vi "Save Wave Data.vi"(10 "Time and Data":T3, 11 "Sample Settings":T1={"设备信息"={"初始索引子集"=[], "模拟信号采集通道"="", "数字-供电"="", "数字-光控"="", "光控设备"="", "光电设备分离？"=FALSE, "光谱保存路径"=path "", "环数"=0}, "测量控制"={"测头拿起"=FALSE, "起始保存"=FALSE, "测头供电"=TRUE, "测头出光"=TRUE}, "测量"={"每波长测量次数"=5, "波长"=[0, 0, 0, 0, 0, 0], "起始周期"=0, "起始测量周期"=0}, "等待"={"等待时间(s)"=0.0, "等待方式"=FALSE, "每x周期/点等待"=8, "等待时"=enum."无电无光"}, "校准"={"暗电流校准值初值"=[], "温度校准值"=[0.0, 0.0, 0.0, 0.0, 0.0, 0.0, 0.00013, 0.00013, 0.00013, 0.00013, 0.00013, 0.00013], "校准模式"=enum."逐周期"}, "图表相关"={"文件-时间"=""}, "CSM"={"CSM Name"=""}}) -> ()   [LabVIEW 2026, in "UI-无创.lvlib" / "Logging.lvlib"]
uses:
  Logging.lvlib
  Supports/Time and Data_OP.ctl
  Supports/Sample Settings.ctl
  <vilib>/Utility/file.llb/Write To Spreadsheet File (DBL).vi
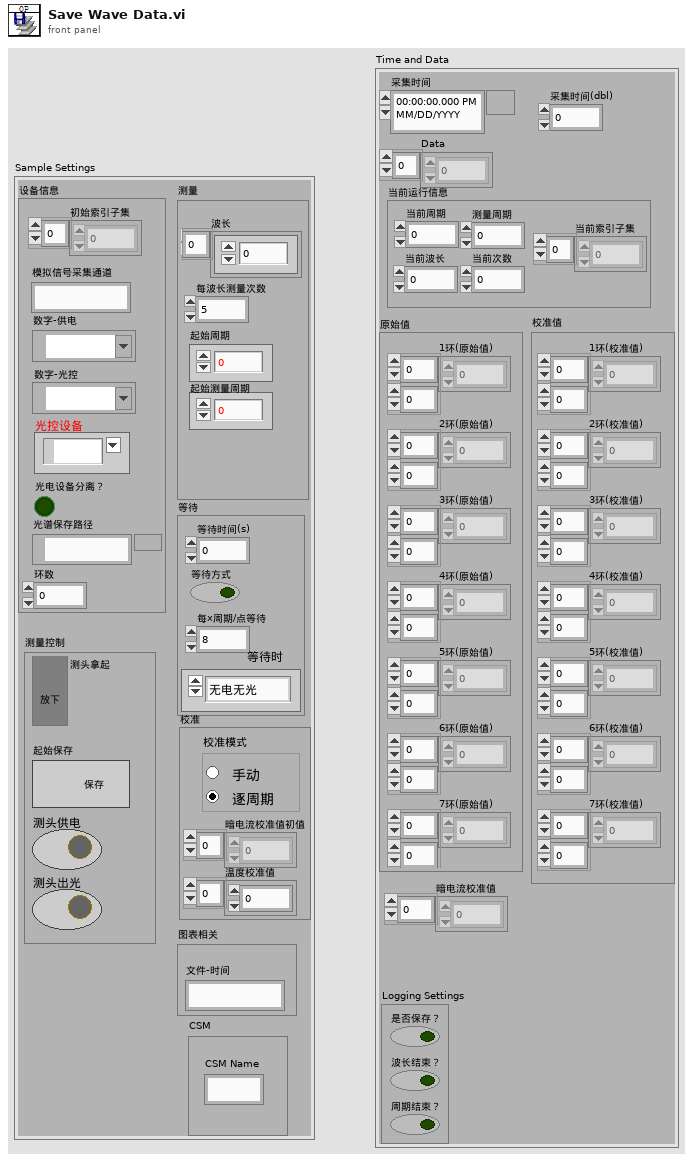
[diagram p1: front panel]
types:
  T1 = typedef "UI-无创.lvlib/Sample Settings.ctl" = cluster{"设备信息":cluster{"初始索引子集":i8[], "模拟信号采集通道":string, "数字-供电":refnum<k21>, "数字-光控":refnum<k21>, "光控设备":tag, "光电设备分离？":bool, "光谱保存路径":path, "环数":u8}, "测量控制":cluster{"测头拿起":bool, "起始保存":bool, "测头供电":bool, "测头出光":bool}, "测量":cluster{"每波长测量次数":i32, "波长":i32[], "起始周期":i32, "起始测量周期":i32}, "等待":cluster{"等待时间(s)":dbl, "等待方式":bool, "每x周期/点等待":i32, "等待时":enum16{"无电无光", "有电无光", "无电有光", "有电有光"}}, "校准":cluster{"暗电流校准值初值":dbl[], "温度校准值":dbl[], "校准模式":T2}, "图表相关":cluster{"文件-时间":string}, "CSM":cluster{"CSM Name":string}}
  T2 = typedef "UI-无创.lvlib/暗电流校准模式.ctl" = enum32{"手动", "逐周期"}
  T3 = typedef "UI-无创.lvlib/Time and Data_OP.ctl" = cluster{"采集时间":timestamp, "采集时间(dbl)":dbl, "Data":dbl[], "当前运行信息":cluster{"当前周期":i32, "当前次数":i32, "测量周期":i32, "当前索引子集":i8[], "当前波长":i32}, "暗电流校准值":dbl[], "Logging Settings":cluster{"是否保存？":bool, "波长结束？":bool, "周期结束？":bool}, "原始值":cluster{"1环(原始值)":dbl[][], "2环(原始值)":dbl[][], "3环(原始值)":dbl[][], "4环(原始值)":dbl[][], "5环(原始值)":dbl[][], "6环(原始值)":dbl[][], "7环(原始值)":dbl[][]}, "校准值":cluster{"1环(校准值)":dbl[][], "2环(校准值)":dbl[][], "3环(校准值)":dbl[][], "4环(校准值)":dbl[][], "5环(校准值)":dbl[][], "6环(校准值)":dbl[][], "7环(校准值)":dbl[][]}}
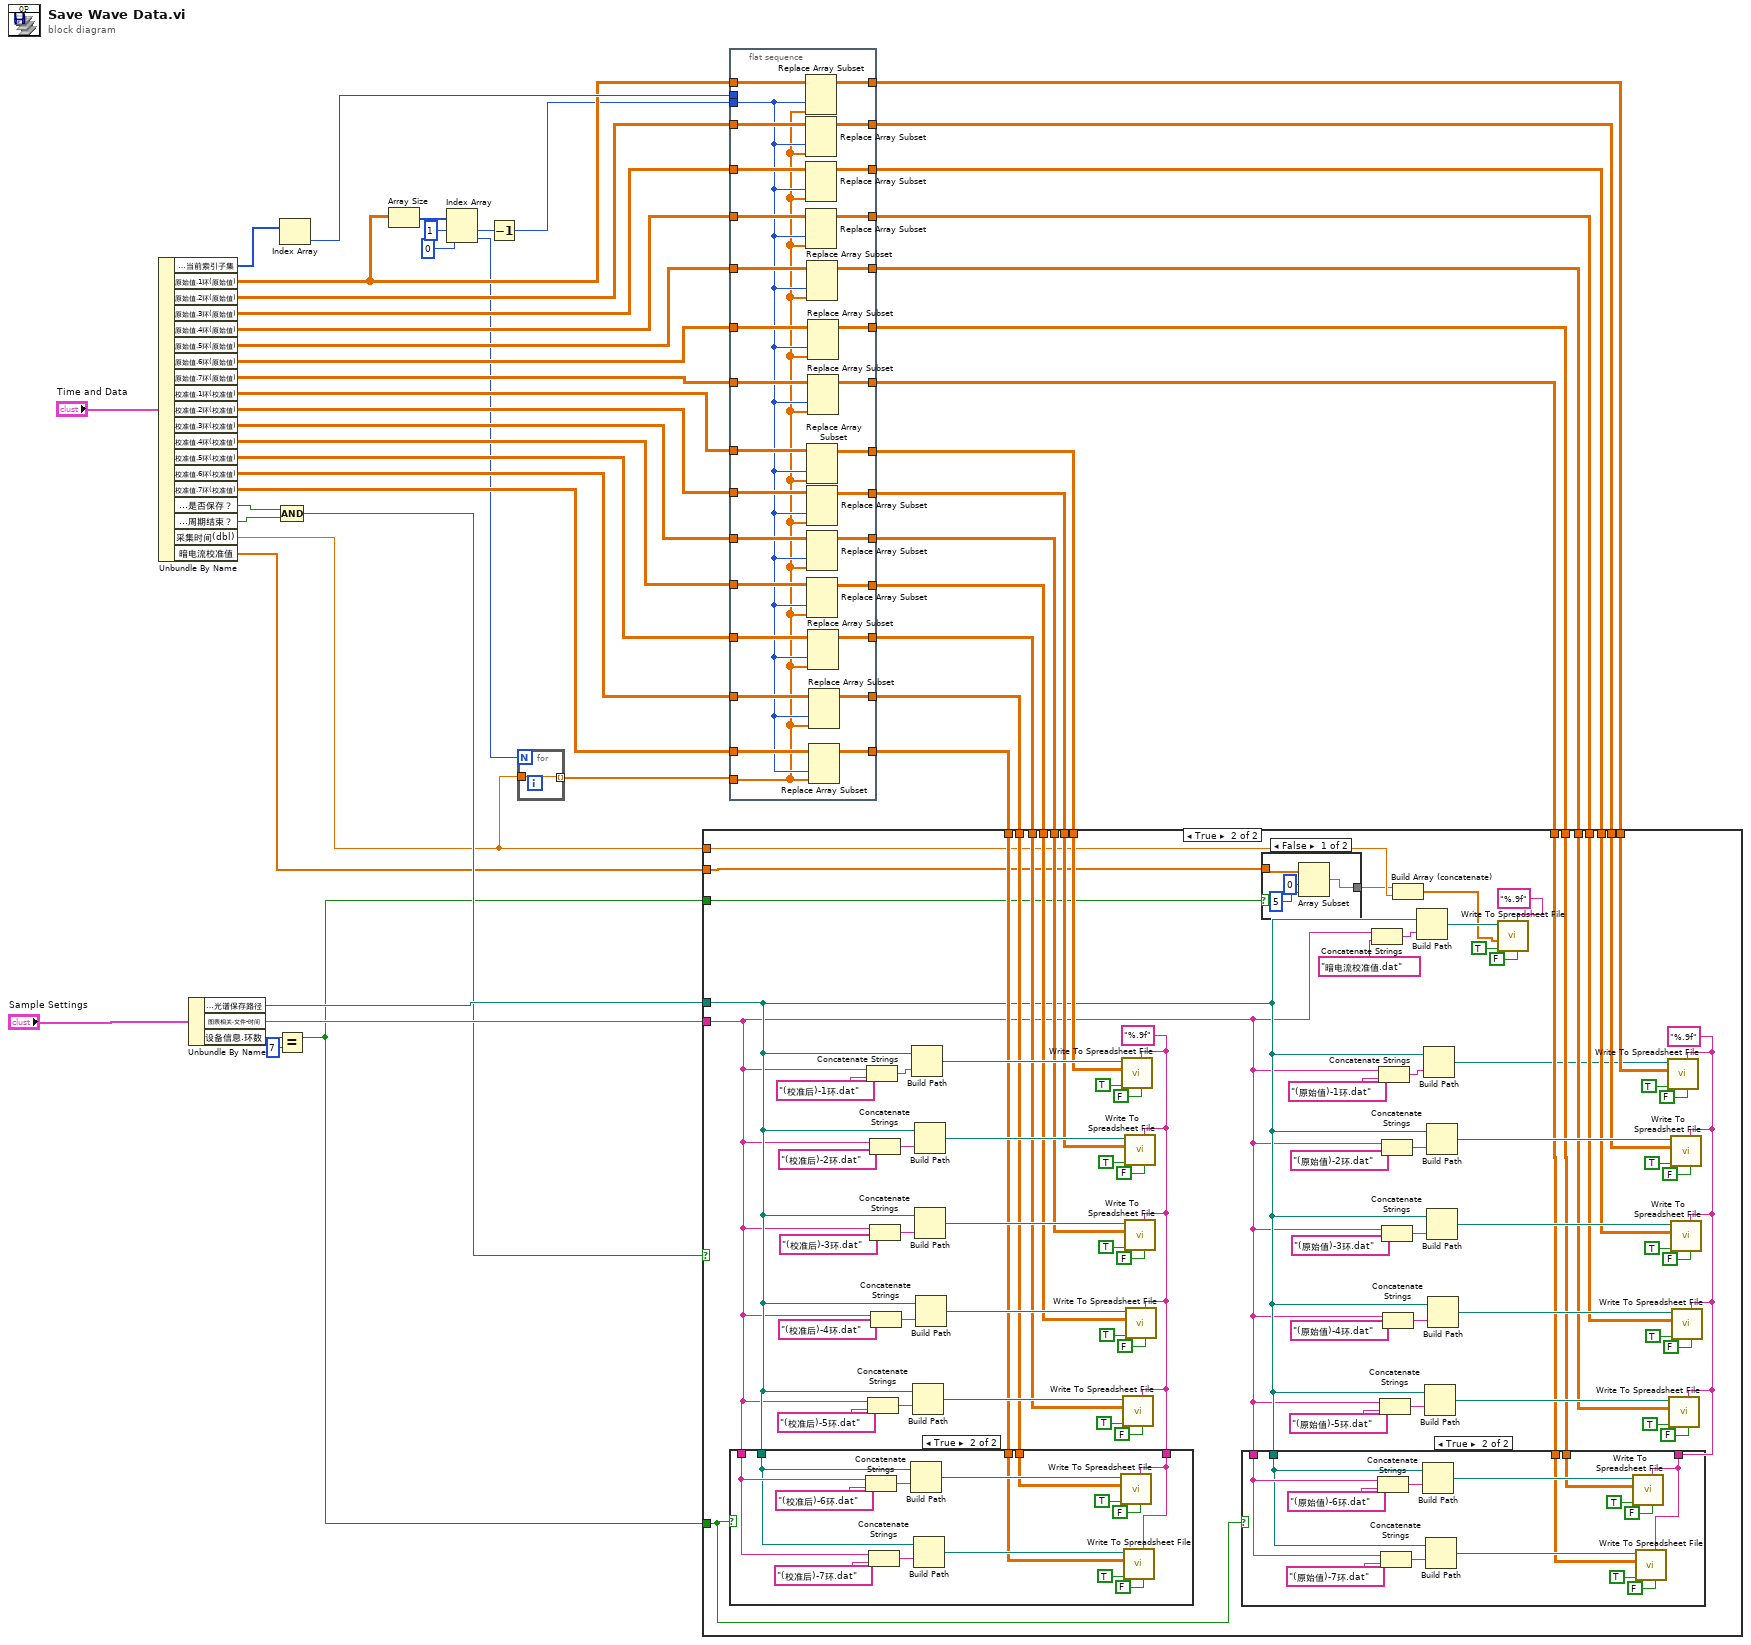
[diagram p0: block diagram]
diagram:
  n1 = Unbundle By Name("Time and Data") -> ("当前运行信息.当前索引子集"=w39:i8[], "原始值.1环(原始值)"=w37:dbl[][], "原始值.2环(原始值)"=w43:dbl[][], "原始值.3环(原始值)"=w42:dbl[][], "原始值.4环(原始值)"=w34:dbl[][], "原始值.5环(原始值)"=w33:dbl[][], "原始值.6环(原始值)"=w32:dbl[][], "原始值.7环(原始值)"=w31:dbl[][], "校准值.1环(校准值)"=w30:dbl[][], "校准值.2环(校准值)"=w28:dbl[][], "校准值.3环(校准值)"=w29:dbl[][], "校准值.4环(校准值)"=w27:dbl[][], "校准值.5环(校准值)"=w26:dbl[][], "校准值.6环(校准值)"=w41:dbl[][], "校准值.7环(校准值)"=w40:dbl[][], "Logging Settings.是否保存？"=w45:bool, "Logging Settings.周期结束？"=w46:bool, "采集时间(dbl)"=w6:dbl, "暗电流校准值"=w9:dbl[])
  n2 = Unbundle By Name("Sample Settings") -> ("设备信息.光谱保存路径"=w48:path, "图表相关.文件-时间"=w47:string, "设备信息.环数"=w8:u8)
  n3 = Equal?(x=w8, y=u8 7) -> (x = y?=w2:bool)
  n4 = Index Array(array=w39) -> (element=w38:i8)  [unwired: 1 in]
  n5 = Compound Arithmetic op=AND ("复合运算")(w45, w46) -> (w44:bool)
  n6 = Array Size(array=w37) -> (size(s)=w36:i32[])
  n7 = Index Array(array=w36, index #1=1 ("索引"), index #2=0 ("索引")) -> (element #1=w10:i32, element #2=w3:i32)
  n8 = Decrement(x=w10) -> (x-1=w25:i32)
  n9 = for "For循环" {
    N: w3 -> [_]
    tunnel: w6 -> [w50]
    tunnel: [w50] -> w5 mode=indexing
  }
  n10 = case shown="True" w44 {
    tunnel: w24 -> [_ w79]
    tunnel: w23 -> [_ w78]
    tunnel: w22 -> [_ w77]
    tunnel: w21 -> [_ w76]
    tunnel: w20 -> [_ w75]
    tunnel: w19 -> [_ w74]
    tunnel: w18 -> [_ w73]
    tunnel: w2 -> [_ w72]
    tunnel: w48 -> [_ w57]
    tunnel: w47 -> [_ w56]
    tunnel: w17 -> [_ w71]
    tunnel: w16 -> [_ w70]
    tunnel: w15 -> [_ w69]
    tunnel: w14 -> [_ w68]
    tunnel: w13 -> [_ w67]
    tunnel: w12 -> [_ w66]
    tunnel: w11 -> [_ w65]
    tunnel: w6 -> [_ w53]
    tunnel: w9 -> [_ w54]
    tunnel: w2 -> [_ w55]
    frame False {
    }
    frame True {
      w80 = "%.9f" ("format (%.3f)")
      w105 = "%.9f" ("format (%.3f)")
      n11 = case shown="True" w72 {
        tunnel: w56 -> [_ w155]
        tunnel: w57 -> [_ w154]
        tunnel: w66 -> [_ w153]
        tunnel: w65 -> [_ w152]
        tunnel: w105 -> [_ w151]
        frame False {
        }
        frame True {
          n12 = Concatenate Strings(w155, "(校准后)-6环.dat" ("字符串")) -> (w164:string)
          n13 = Concatenate Strings(w155, "(校准后)-7环.dat" ("字符串")) -> (w159:string)
          n14 = Build Path(base path=w154, name or relative path=w164) -> (appended path=w165:path)
          n15 = Build Path(base path=w154, name or relative path=w159) -> (appended path=w160:path)
          n16 = call-poly <vilib>:"Write To Spreadsheet File.vi"("transpose? (no:F)"=FALSE, "format (%.3f)"=w151, "append to file? (new file:F)"=TRUE, "2D data"=w153, "file path (dialog if empty)"=w165) -> ()  [unwired: 3 in, 1 out]
          n17 = call-poly <vilib>:"Write To Spreadsheet File.vi"("transpose? (no:F)"=FALSE, "format (%.3f)"=w151, "append to file? (new file:F)"=TRUE, "2D data"=w152, "file path (dialog if empty)"=w160) -> ()  [unwired: 3 in, 1 out]
        }
      }
      n18 = Concatenate Strings(w56, "(校准后)-1环.dat" ("字符串")) -> (w129:string)
      n19 = Concatenate Strings(w56, "(校准后)-5环.dat" ("字符串")) -> (w109:string)
      n20 = Concatenate Strings(w56, "(校准后)-2环.dat" ("字符串")) -> (w122:string)
      n21 = Concatenate Strings(w56, "(校准后)-3环.dat" ("字符串")) -> (w119:string)
      n22 = Concatenate Strings(w56, "(校准后)-4环.dat" ("字符串")) -> (w112:string)
      n23 = Build Path(base path=w57, name or relative path=w129) -> (appended path=w130:path)
      n24 = Build Path(base path=w57, name or relative path=w109) -> (appended path=w110:path)
      n25 = Build Path(base path=w57, name or relative path=w122) -> (appended path=w121:path)
      n26 = Build Path(base path=w57, name or relative path=w119) -> (appended path=w120:path)
      n27 = Build Path(base path=w57, name or relative path=w112) -> (appended path=w111:path)
      n28 = call-poly <vilib>:"Write To Spreadsheet File.vi"("transpose? (no:F)"=FALSE, "format (%.3f)"=w105, "append to file? (new file:F)"=TRUE, "2D data"=w71, "file path (dialog if empty)"=w130) -> ()  [unwired: 3 in, 1 out]
      n29 = call-poly <vilib>:"Write To Spreadsheet File.vi"("transpose? (no:F)"=FALSE, "format (%.3f)"=w105, "append to file? (new file:F)"=TRUE, "2D data"=w67, "file path (dialog if empty)"=w110) -> ()  [unwired: 3 in, 1 out]
      n30 = call-poly <vilib>:"Write To Spreadsheet File.vi"("transpose? (no:F)"=FALSE, "format (%.3f)"=w105, "append to file? (new file:F)"=TRUE, "2D data"=w70, "file path (dialog if empty)"=w121) -> ()  [unwired: 3 in, 1 out]
      n31 = call-poly <vilib>:"Write To Spreadsheet File.vi"("transpose? (no:F)"=FALSE, "format (%.3f)"=w105, "append to file? (new file:F)"=TRUE, "2D data"=w69, "file path (dialog if empty)"=w120) -> ()  [unwired: 3 in, 1 out]
      n32 = call-poly <vilib>:"Write To Spreadsheet File.vi"("transpose? (no:F)"=FALSE, "format (%.3f)"=w105, "append to file? (new file:F)"=TRUE, "2D data"=w68, "file path (dialog if empty)"=w111) -> ()  [unwired: 3 in, 1 out]
      n33 = case shown="True" w72 {
        tunnel: w56 -> [_ w140]
        tunnel: w57 -> [_ w139]
        tunnel: w74 -> [_ w138]
        tunnel: w73 -> [_ w137]
        tunnel: w80 -> [_ w136]
        frame False {
        }
        frame True {
          n34 = Concatenate Strings(w140, "(原始值)-6环.dat" ("字符串")) -> (w149:string)
          n35 = Concatenate Strings(w140, "(原始值)-7环.dat" ("字符串")) -> (w144:string)
          n36 = Build Path(base path=w139, name or relative path=w149) -> (appended path=w150:path)
          n37 = Build Path(base path=w139, name or relative path=w144) -> (appended path=w145:path)
          n38 = call-poly <vilib>:"Write To Spreadsheet File.vi"("transpose? (no:F)"=FALSE, "format (%.3f)"=w136, "append to file? (new file:F)"=TRUE, "2D data"=w138, "file path (dialog if empty)"=w150) -> ()  [unwired: 3 in, 1 out]
          n39 = call-poly <vilib>:"Write To Spreadsheet File.vi"("transpose? (no:F)"=FALSE, "format (%.3f)"=w136, "append to file? (new file:F)"=TRUE, "2D data"=w137, "file path (dialog if empty)"=w145) -> ()  [unwired: 3 in, 1 out]
        }
      }
      n40 = case shown="False" w55 {
        tunnel: w54 -> [w134 w135]
        tunnel: [w133 w135] -> w51
        frame False {
          n41 = Array Subset(array=w134, index=0 ("索引"), length=5 ("长度")) -> (w133:dbl[])
        }
        frame True {
        }
      }
      n42 = Concatenate Strings(w56, "暗电流校准值.dat" ("字符串")) -> (w60:string)
      n43 = Concatenate Strings(w56, "(原始值)-1环.dat" ("字符串")) -> (w104:string)
      n44 = Concatenate Strings(w56, "(原始值)-5环.dat" ("字符串")) -> (w84:string)
      n45 = Concatenate Strings(w56, "(原始值)-2环.dat" ("字符串")) -> (w97:string)
      n46 = Concatenate Strings(w56, "(原始值)-3环.dat" ("字符串")) -> (w94:string)
      n47 = Concatenate Strings(w56, "(原始值)-4环.dat" ("字符串")) -> (w87:string)
      n48 = Build Array (concatenate)(w51, w53) -> (w52:dbl[])
      n49 = Build Path(base path=w57, name or relative path=w60) -> (appended path=w58:path)
      n50 = Build Path(base path=w57, name or relative path=w104) -> (appended path=w64:path)
      n51 = Build Path(base path=w57, name or relative path=w84) -> (appended path=w85:path)
      n52 = Build Path(base path=w57, name or relative path=w97) -> (appended path=w96:path)
      n53 = Build Path(base path=w57, name or relative path=w94) -> (appended path=w95:path)
      n54 = Build Path(base path=w57, name or relative path=w87) -> (appended path=w86:path)
      n55 = call-poly <vilib>:"Write To Spreadsheet File.vi"("transpose? (no:F)"=FALSE, "format (%.3f)"="%.9f", "append to file? (new file:F)"=TRUE, "1D data"=w52, "file path (dialog if empty)"=w58) -> ()  [unwired: 3 in, 1 out]
      n56 = call-poly <vilib>:"Write To Spreadsheet File.vi"("transpose? (no:F)"=FALSE, "format (%.3f)"=w80, "append to file? (new file:F)"=TRUE, "2D data"=w79, "file path (dialog if empty)"=w64) -> ()  [unwired: 3 in, 1 out]
      n57 = call-poly <vilib>:"Write To Spreadsheet File.vi"("transpose? (no:F)"=FALSE, "format (%.3f)"=w80, "append to file? (new file:F)"=TRUE, "2D data"=w75, "file path (dialog if empty)"=w85) -> ()  [unwired: 3 in, 1 out]
      n58 = call-poly <vilib>:"Write To Spreadsheet File.vi"("transpose? (no:F)"=FALSE, "format (%.3f)"=w80, "append to file? (new file:F)"=TRUE, "2D data"=w78, "file path (dialog if empty)"=w96) -> ()  [unwired: 3 in, 1 out]
      n59 = call-poly <vilib>:"Write To Spreadsheet File.vi"("transpose? (no:F)"=FALSE, "format (%.3f)"=w80, "append to file? (new file:F)"=TRUE, "2D data"=w77, "file path (dialog if empty)"=w95) -> ()  [unwired: 3 in, 1 out]
      n60 = call-poly <vilib>:"Write To Spreadsheet File.vi"("transpose? (no:F)"=FALSE, "format (%.3f)"=w80, "append to file? (new file:F)"=TRUE, "2D data"=w76, "file path (dialog if empty)"=w86) -> ()  [unwired: 3 in, 1 out]
    }
  }
  n61 = flat-sequence {
    tunnel: w43 -> [w195]
    tunnel: w42 -> [w194]
    tunnel: w41 -> [w193]
    tunnel: w40 -> [w192]
    tunnel: w5 -> [w166]
    tunnel: w38 -> [_]
    tunnel: w37 -> [w191]
    tunnel: w34 -> [w190]
    tunnel: w33 -> [w189]
    tunnel: w32 -> [w188]
    tunnel: w31 -> [w187]
    tunnel: w30 -> [w186]
    tunnel: w29 -> [w185]
    tunnel: w28 -> [w184]
    tunnel: w27 -> [w183]
    tunnel: w26 -> [w182]
    tunnel: w25 -> [w181]
    tunnel: [w180] -> w24
    tunnel: [w179] -> w23
    tunnel: [w178] -> w22
    tunnel: [w177] -> w21
    tunnel: [w176] -> w20
    tunnel: [w175] -> w19
    tunnel: [w174] -> w18
    tunnel: [w173] -> w17
    tunnel: [w172] -> w16
    tunnel: [w171] -> w15
    tunnel: [w170] -> w14
    tunnel: [w169] -> w13
    tunnel: [w168] -> w12
    tunnel: [w167] -> w11
    frame #0 {
      n62 = Replace Array Subset(array=w191, new element=w166, index (col)=w181) -> (w180:dbl[][])  [unwired: 1 in]
      n63 = Replace Array Subset(array=w195, new element=w166, index (col)=w181) -> (w179:dbl[][])  [unwired: 1 in]
      n64 = Replace Array Subset(array=w194, new element=w166, index (col)=w181) -> (w178:dbl[][])  [unwired: 1 in]
      n65 = Replace Array Subset(array=w190, new element=w166, index (col)=w181) -> (w177:dbl[][])  [unwired: 1 in]
      n66 = Replace Array Subset(array=w189, new element=w166, index (col)=w181) -> (w176:dbl[][])  [unwired: 1 in]
      n67 = Replace Array Subset(array=w186, new element=w166, index (col)=w181) -> (w173:dbl[][])  [unwired: 1 in]
      n68 = Replace Array Subset(array=w184, new element=w166, index (col)=w181) -> (w172:dbl[][])  [unwired: 1 in]
      n69 = Replace Array Subset(array=w185, new element=w166, index (col)=w181) -> (w171:dbl[][])  [unwired: 1 in]
      n70 = Replace Array Subset(array=w183, new element=w166, index (col)=w181) -> (w170:dbl[][])  [unwired: 1 in]
      n71 = Replace Array Subset(array=w188, new element=w166, index (col)=w181) -> (w175:dbl[][])  [unwired: 1 in]
      n72 = Replace Array Subset(array=w187, new element=w166, index (col)=w181) -> (w174:dbl[][])  [unwired: 1 in]
      n73 = Replace Array Subset(array=w182, new element=w166, index (col)=w181) -> (w169:dbl[][])  [unwired: 1 in]
      n74 = Replace Array Subset(array=w193, new element=w166, index (col)=w181) -> (w168:dbl[][])  [unwired: 1 in]
      n75 = Replace Array Subset(array=w192, new element=w166, index (col)=w181) -> (w167:dbl[][])  [unwired: 1 in]
    }
  }
